vi "Send Return Value.vi"(8 "error in (no error)":errorcluster, 10 "Return Value":variant, 11 "Call in":refnum<class "Call.lvclass">) -> (0 "error out":errorcluster)   [LabVIEW 2020, in "jki_python_bridge.lvlib" / "Call.lvclass"]
uses:
  Call.lvclass
  Server/Type Definitions/Python Response - Cluster.ctl
  Call.lvclass/Call.ctl
  Server/Server.lvclass
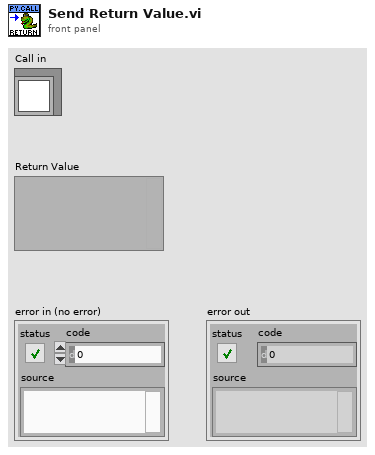
[diagram p1: front panel]
types:
  T1 = typedef "jki_python_bridge.lvlib/Server.lvclass/Python Response - Cluster.ctl" = cluster{"Python Response":variant, "error out":errorcluster}
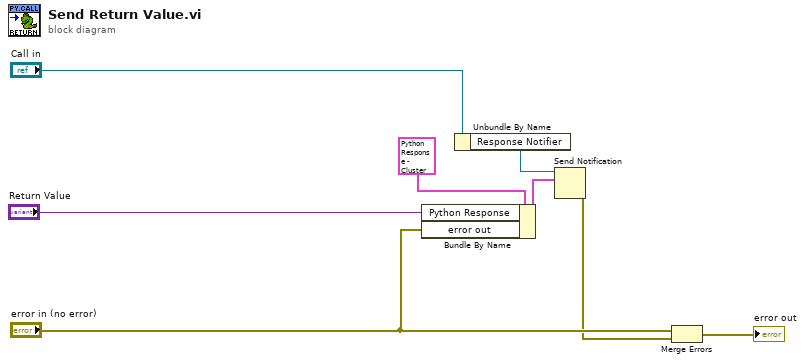
[diagram p0: block diagram]
diagram:
  n1 = Bundle By Name(cluster=T1 {"Python Response"=variant, "error out"={"status"=FALSE, "code"=0, "source"=""}} ("Python Response"), "Python Response"="Return Value", "error out"="error in (no error)") -> (w4:T1)
  n2 = Unbundle By Name("Call in") -> ("Response Notifier"=w2:refnum<notifier>)
  n3 = Send Notification(notification=w4, notifier=w2) -> (error out=w1:errorcluster)  [unwired: 1 in, 1 out]
  n4 = Merge Errors("error in (no error)", w1) -> (→"error out":errorcluster)
